vi "Level_Setup.vi"(0 "State":T1={"Tick"=0, "Phase"=0, "PhaseTicks"=0, "Level"=1, "Room"=0, "X10"=0, "Y10"=0, "VY10"=0, "Mode"=0, "Facing"=0, "Run"=0, "Vert"=0, "StandY"=0, "EntryX10"=0, "EntryY10"=0, "EntryMode"=0, "Lives"=4, "Score"=0, "NextLife"=10000, "KeyR"=0, "KeyB"=0, "KeyY"=0, "Torch"=FALSE, "FloorPhase"=0, "Dead"=FALSE, "LevelStart"=FALSE, "Quit"=FALSE, "Sound"=0, "Seed"=12345, "DemoStep"=0, "Tiles"=[], "World"=[], "Enemies"=[], "Highscores"=[], "Name"=[0, 0, 0], "Cursor"=0}, 5 "Rooms":T2(array[cluster]), 7 "Level":i32=1, 11 "error in":errorcluster) -> (4 "State out":T1={"Tick"=0, "Phase"=0, "PhaseTicks"=0, "Level"=1, "Room"=0, "X10"=0, "Y10"=0, "VY10"=0, "Mode"=0, "Facing"=0, "Run"=0, "Vert"=0, "StandY"=0, "EntryX10"=0, "EntryY10"=0, "EntryMode"=0, "Lives"=4, "Score"=0, "NextLife"=10000, "KeyR"=0, "KeyB"=0, "KeyY"=0, "Torch"=FALSE, "FloorPhase"=0, "Dead"=FALSE, "LevelStart"=FALSE, "Quit"=FALSE, "Sound"=0, "Seed"=12345, "DemoStep"=0, "Tiles"=[], "World"=[], "Enemies"=[], "Highscores"=[], "Name"=[0, 0, 0], "Cursor"=0}, 15 "error out":errorcluster)   [LabVIEW 2020, in "GH_Engine.lvlib"]
doc: "Starts a level: all rooms as they are in the files (World = Rooms), Claude on the start tile P of the first room, no keys, no torch, enemies of the first room, phase Ready with the LEVEL message. Score, lives and highscores stay."
uses:
  GH_Engine.lvlib
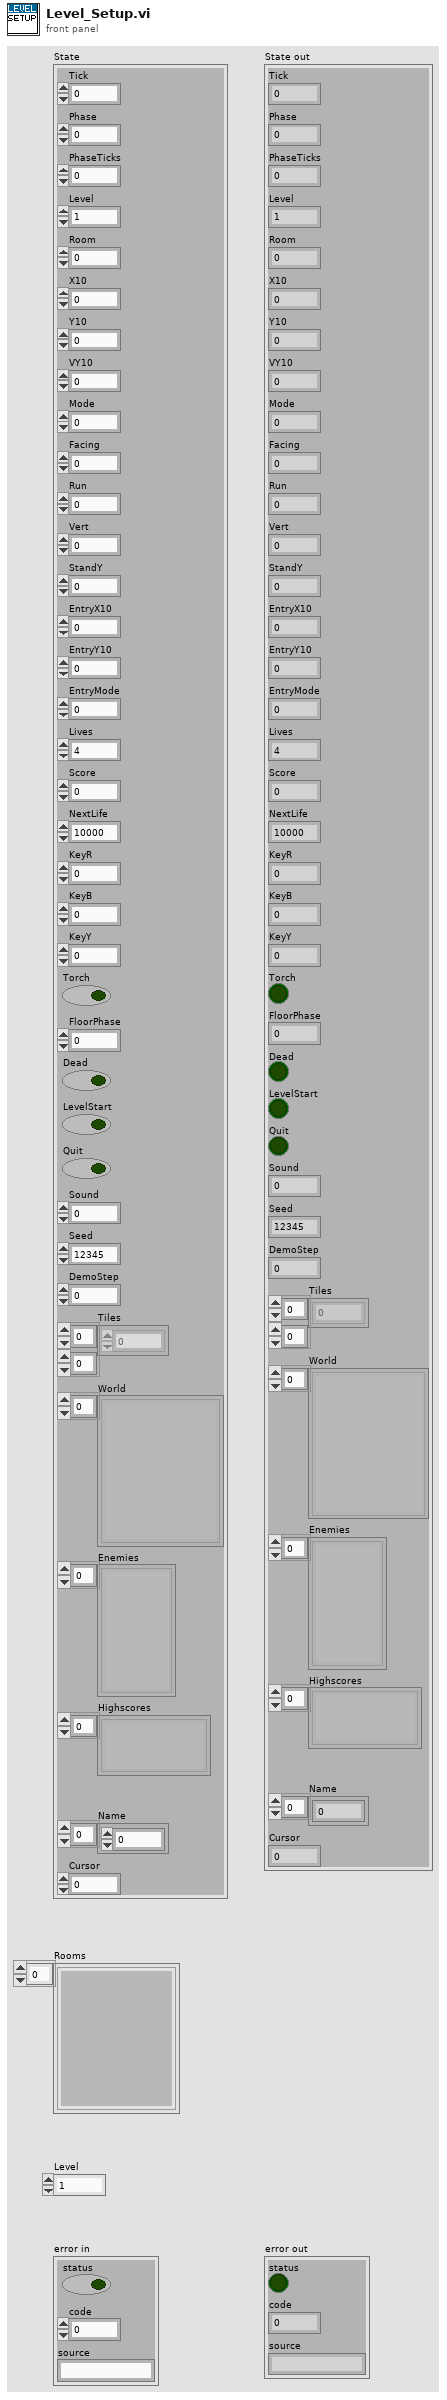
[diagram p1: front panel]
types:
  T1 = cluster{"Tick":u32, "Phase":i32, "PhaseTicks":i32, "Level":i32, "Room":i32, "X10":i32, "Y10":i32, "VY10":i32, "Mode":i32, "Facing":i32, "Run":i32, "Vert":i32, "StandY":i32, "EntryX10":i32, "EntryY10":i32, "EntryMode":i32, "Lives":i32, "Score":i32, "NextLife":i32, "KeyR":i32, "KeyB":i32, "KeyY":i32, "Torch":bool, "FloorPhase":i32, "Dead":bool, "LevelStart":bool, "Quit":bool, "Sound":i32, "Seed":u32, "DemoStep":i32, "Tiles":u8[][], "World":cluster{"ID":string, "Depth":i32, "Column":i32, "Tiles":u8[][]}[], "Enemies":cluster{"Kind":i32, "X10":i32, "Y10":i32, "Dir":i32, "Mode":i32}[], "Highscores":cluster{"Score":i32, "Name":string}[], "Name":i32[], "Cursor":i32}
  T2 = cluster{"ID":string, "Depth":i32, "Column":i32, "Tiles":u8[][]}[]
  T3 = cluster{"ID":string, "Depth":i32, "Column":i32, "Tiles":u8[][]}
  T4 = cluster{"Kind":i32, "X10":i32, "Y10":i32, "Dir":i32, "Mode":i32}[]
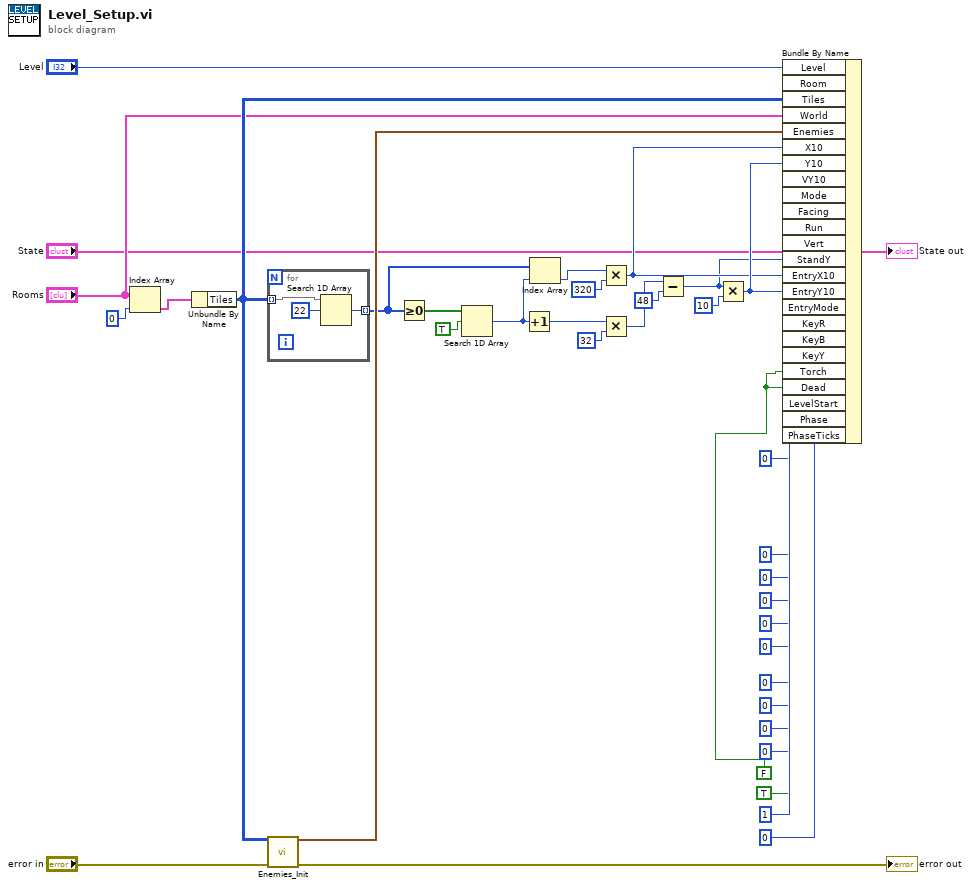
[diagram p0: block diagram]
diagram:
  w24 = FALSE
  n1 = Index Array(array="Rooms", index=0) -> (element=w6:T3)
  n2 = Unbundle By Name(w6) -> ("Tiles"=w7:u8[][])
  n3 = for {
    tunnel: w7 -> [w39] mode=indexing
    tunnel: [w41] -> w8 mode=indexing
    n4 = Search 1D Array(1D array=w39, element=u8 22) -> (index of element=w41:i32)  [unwired: 1 in]
  }
  n5 = call "Enemies_Init.vi"("Tiles"=w7, "error in"="error in") -> ("Enemies"=w22:T4, "error out"=→"error out":errorcluster)  [unwired: 12 in]
  n6 = Greater Or Equal To 0?(x=w8) -> (x >= 0?=w9:bool[])
  n7 = Search 1D Array(1D array=w9, element=TRUE) -> (index of element=w11:i32)  [unwired: 1 in]
  n8 = Increment(x=w11) -> (x+1=w13:i32)
  n9 = Index Array(array=w8, index=w11) -> (element=w12:i32)
  n10 = Multiply(x=w12, y=320) -> (x*y=w19:i32)
  n11 = Multiply(x=w13, y=32) -> (x*y=w15:i32)
  n12 = Subtract(x=w15, y=48) -> (x-y=w17:i32)
  n13 = Multiply(x=w17, y=10) -> (x*y=w21:i32)
  n14 = Bundle By Name(cluster="State", "Level"="Level", "Room"=0, "Tiles"=w7, "World"="Rooms", "Enemies"=w22, "X10"=w19, "Y10"=w21, "VY10"=0, "Mode"=0, "Facing"=0, "Run"=0, "Vert"=0, "StandY"=w17, "EntryX10"=w19, "EntryY10"=w21, "EntryMode"=0, "KeyR"=0, "KeyB"=0, "KeyY"=0, "Torch"=w24, "Dead"=w24, "LevelStart"=TRUE, "Phase"=1, "PhaseTicks"=0) -> (→"State out":T1)
